vi "Get Filter Arguments Reference.vi"(11 "滤波参数引用":refnum<vi>) -> (0 "参数2":refnum<vi>, 1 "参数1":refnum<vi>, 2 "滤波方式":refnum<vi>, 3 "滤波器类型":refnum<vi>)   [LabVIEW 2020, in "Data Viewer.lvlib" / "Data Viewer.lvclass"]
uses:
  Data Viewer.lvclass
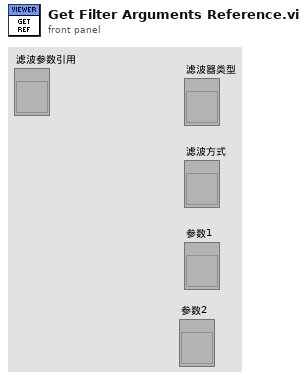
[diagram p1: front panel]
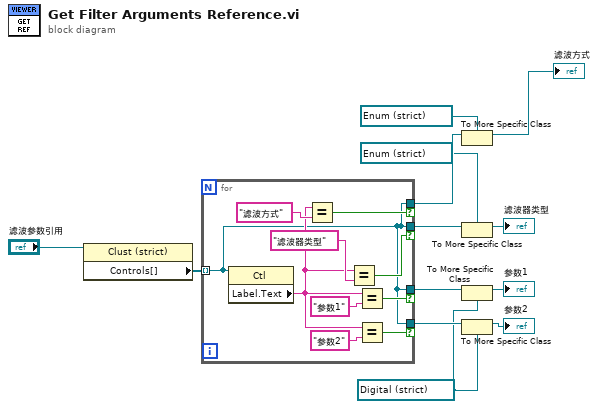
[diagram p0: block diagram]
diagram:
  w10 = refnum<vi> refnum ("参数1")
  n1 = property class="Clust (strict)"(reference="滤波参数引用") -> ("Controls[]"=w3:refnum<vi>[])  [unwired: 1 in, 2 out]
  n2 = for {
    tunnel: w3 -> [w15] mode=indexing
    tunnel: [w15] -> w4 if=w22
    tunnel: [w15] -> w8 if=w20
    tunnel: [w15] -> w9 if=w18
    tunnel: [w15] -> w11 if=w14
    n3 = property class="Ctl"(reference=w15) -> ("Label.Text"=w16:string)  [unwired: 1 in, 2 out]
    n4 = Equal?(x=w16, y="滤波方式") -> (x = y?=w20:bool)
    n5 = Equal?(x=w16, y="滤波器类型") -> (x = y?=w22:bool)
    n6 = Equal?(x=w16, y="参数1") -> (x = y?=w18:bool)
    n7 = Equal?(x=w16, y="参数2") -> (x = y?=w14:bool)
  }
  n8 = To More Specific Class(target class=refnum<vi> refnum ("枚举"), reference=w8) -> (specific class reference=→"滤波方式":refnum<vi>)  [unwired: 1 in, 1 out]
  n9 = To More Specific Class(target class=refnum<vi> refnum ("滤波器类型"), reference=w4) -> (specific class reference=→"滤波器类型":refnum<vi>)  [unwired: 1 in, 1 out]
  n10 = To More Specific Class(target class=w10, reference=w9) -> (specific class reference=→"参数1":refnum<vi>)  [unwired: 1 in, 1 out]
  n11 = To More Specific Class(target class=w10, reference=w11) -> (specific class reference=→"参数2":refnum<vi>)  [unwired: 1 in, 1 out]
